vi "Command Type.vi"(11 "Numeric Command Config in":refnum<class "Numeric Command Config.lvclass">) -> (2 "Command Type":T1)   [LabVIEW 2020, in "VolatusSeqConfig.lvlib" / "Numeric Command Config.lvclass"]
uses:
  Numeric Command Config.lvclass
  Numeric Command Config.lvclass/Numeric Command Config.ctl
  Command Type.ctl
  VolatusSeqConfig.lvlib
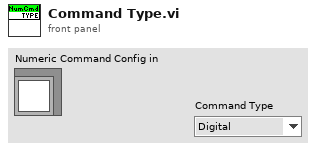
[diagram p1: front panel]
types:
  T1 = typedef "VolatusSeqConfig.lvlib/Command Type.ctl" = enum16{"Digital", "Numeric", "Transition", "Stop Seq", "Start Log", "Stop Log"}
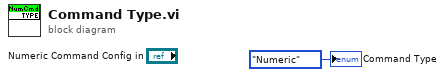
[diagram p0: block diagram]
diagram:
  "Command Type" <- Command_Type."Numeric" ("Command Type")
